vi "MB_WriteCoil.vi"(0 "connection ID":refnum<k5>, 1 "Address":u16, 2 "Value":bool, 3 "error in (no error)":errorcluster) -> (5 "connection ID out":refnum<k5>, 7 "error out":errorcluster)   [LabVIEW 2018]
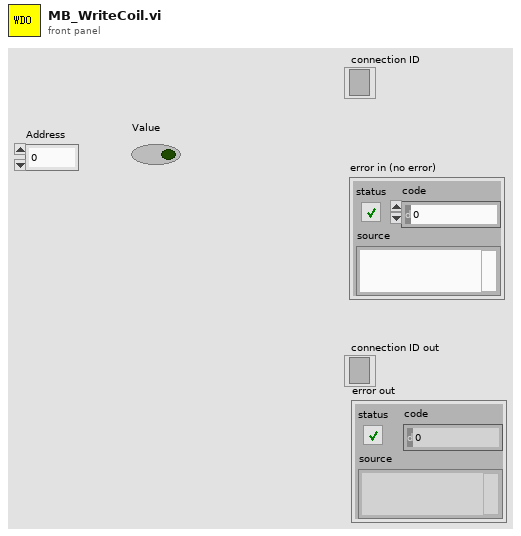
[diagram p1: front panel]
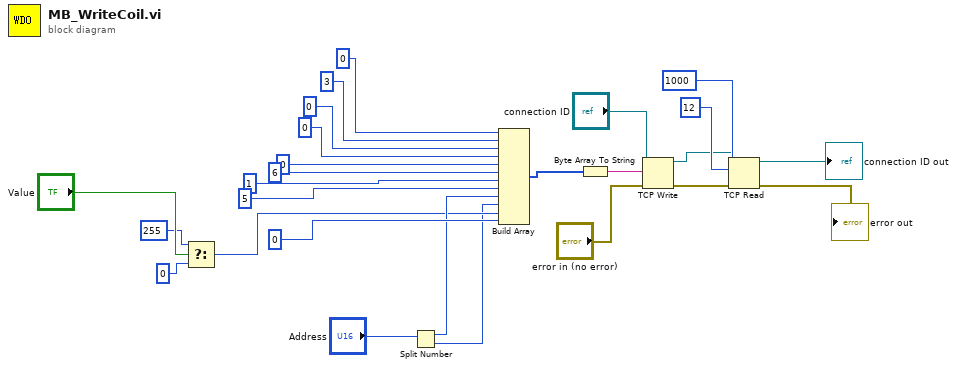
[diagram p0: block diagram]
diagram:
  n1 = Select(t=u8 255, s="Value", f=u8 0) -> (s? t:f=w12:u8)
  n2 = Split Number(x="Address") -> (hi(x)=w13:u8, lo(x)=w11:u8)
  n3 = Build Array(u8 0, u8 3, u8 0, u8 0, u8 0 ("element"), u8 6, u8 1 ("element"), u8 5, w13, w11, w12, u8 0 ("element")) -> (w10:u8[])
  n4 = Byte Array To String(unsigned byte array=w10) -> (string=w9:string)
  n5 = TCP Write(connection ID="connection ID", data in=w9, error in (no error)="error in (no error)") -> (connection ID out=w6:refnum<k5>, error out=w5:errorcluster)  [unwired: 1 in, 1 out]
  n6 = TCP Read(connection ID=w6, bytes to read=12, error in (no error)=w5, 9:1000 ("timeout ms (25000)")) -> (connection ID out=→"connection ID out":refnum<k5>, error out=→"error out":errorcluster)  [unwired: 1 in, 1 out]
